vi "fake tool error descriptions.vi"(8 "error in (no error)":errorcluster, 11 "previous error":errorcluster) -> (0 "error out":errorcluster, 3 "last error":errorcluster)   [LabVIEW 2020, in "MCP Server tests.lvlib"]
doc: "Fake tool to test that tools/list leaves out LabVIEW's default error cluster descriptions. error in (no error) and error out carry the descriptions of NI's Error In 3D and Error Out 3D controls, elements included. previous error and last error carry descriptions of their own (previous error also on its source element, last error on its code element) and NI's defaults on their other elements. Each input is returned unchanged on an output."
uses:
  MCP Server tests.lvlib
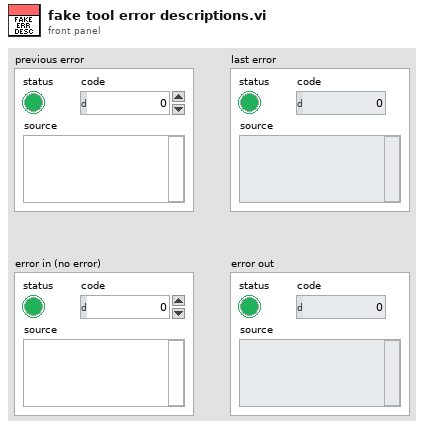
[diagram p1: front panel]
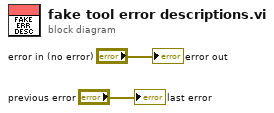
[diagram p0: block diagram]
diagram:
  "last error" <- "previous error"
  "error out" <- "error in (no error)"
